vi "Parse CIF PCAP Config Custom Data.vi"(7 "offset in":i32, 11 "Flattened PCAP FIFO Custom Data":u8[](array[numeric])) -> (2 "Linktype Name":string, 3 "LinkType":u32, 5 "offset out":i32)   [LabVIEW 2021, in "Iceoryx Channel Utilities.lvlib"]
uses:
  Iceoryx Channel Utilities.lvlib
  <vilib>/CIF Foundation/CIF Utilities/DataTypes/DataTypes_CIF_U.lvlib
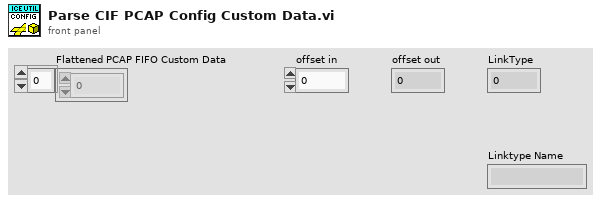
[diagram p1: front panel]
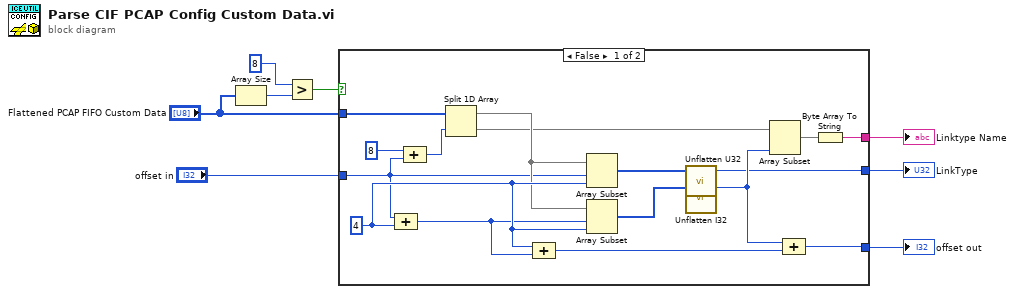
[diagram p0: block diagram]
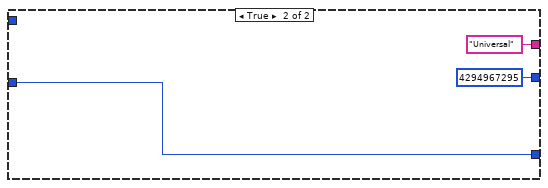
[diagram p2: hidden frame]
diagram:
  n1 = Array Size(array="Flattened PCAP FIFO Custom Data") -> (size(s)=w6:i32)
  n2 = Greater?(x=8, y=w6) -> (0:w4:bool)
  n3 = case shown="False" w4 {
    tunnel: "offset in" -> [w18 w25]
    tunnel: [w15 w25] -> w7
    tunnel: "Flattened PCAP FIFO Custom Data" -> [w21 _]
    tunnel: [w11 u32 4294967295 ("U32")] -> w2
    tunnel: [w9 "Universal" ("string")] -> w1
    frame False {
      w22 = 4 ("length")
      n4 = Compound Arithmetic op=ADD(w18, w22) -> (w14:i32)
      n5 = Compound Arithmetic op=ADD(8 ("value"), w18) -> (w19:i32)
      n6 = Split 1D Array(array=w21, index=w19) -> (first subarray=w20:u8[], second subarray=w13:u8[])
      n7 = Compound Arithmetic op=ADD(w22, w14) -> (w16:i32)
      n8 = Array Subset(array=w20, index=w18, length=w22) -> (w24:u8[])
      n9 = Array Subset(array=w20, index=w14, length=w22) -> (w23:u8[])
      n10 = call <vilib>:"Unflatten U32.vi"("Flat Data"=w24) -> ("U32"=w11:u32)  [unwired: 4 in]
      n11 = call <vilib>:"Unflatten I32.vi"("Flat Data"=w23) -> ("I32"=w12:i32)  [unwired: 4 in]
      n12 = Array Subset(array=w13, length=w12) -> (w10:u8[])  [unwired: 1 in]
      n13 = Compound Arithmetic op=ADD(w12, w16) -> (w15:i32)
      n14 = Byte Array To String(unsigned byte array=w10) -> (string=w9:string)
    }
    frame True {
    }
  }
  "offset out" <- w7
  "LinkType" <- w2
  "Linktype Name" <- w1
